vi "Dlg_Settings.vi"(0 "Settings":T1={"Sample Rate (Hz)"=1000.0, "Samples per Channel"=100, "Chassis 1 Channels"="cDAQ1Mod1/ai0:7,cDAQ1Mod2/ai0:7,cDAQ1Mod3/ai0:7,cDAQ1Mod4/ai0:7,cDAQ1Mod5/ai0:7,cDAQ1Mod6/ai0:7,cDAQ1Mod7/ai0:7,cDAQ1Mod8/ai0:7", "Chassis 2 Channels"="cDAQ2Mod1/ai0:7,cDAQ2Mod2/ai0:7,cDAQ2Mod3/ai0:7,cDAQ2Mod4/ai0:7,cDAQ2Mod5/ai0:7,cDAQ2Mod6/ai0:7,cDAQ2Mod7/ai0:7,cDAQ2Mod8/ai0:7", "Save Folder"=path "C:/LV_Test/AI DAQ md test/Data"}, 11 "error in":errorcluster) -> (4 "Settings out":T1={"Sample Rate (Hz)"=1000.0, "Samples per Channel"=100, "Chassis 1 Channels"="cDAQ1Mod1/ai0:7,cDAQ1Mod2/ai0:7,cDAQ1Mod3/ai0:7,cDAQ1Mod4/ai0:7,cDAQ1Mod5/ai0:7,cDAQ1Mod6/ai0:7,cDAQ1Mod7/ai0:7,cDAQ1Mod8/ai0:7", "Chassis 2 Channels"="cDAQ2Mod1/ai0:7,cDAQ2Mod2/ai0:7,cDAQ2Mod3/ai0:7,cDAQ2Mod4/ai0:7,cDAQ2Mod5/ai0:7,cDAQ2Mod6/ai0:7,cDAQ2Mod7/ai0:7,cDAQ2Mod8/ai0:7", "Save Folder"=path "C:/LV_Test/AI DAQ md test/Data"}, 6 "OK?":bool, 15 "error out":errorcluster)   [LabVIEW 2026]
doc: "측정 옵션 팝업: 샘플링 속도, 채널당 샘플 수, 섀시별 물리 채널, 저장 폴더. 확인이면 OK? = True."
panel:
  in  "취소":bool
  in  "확인":bool
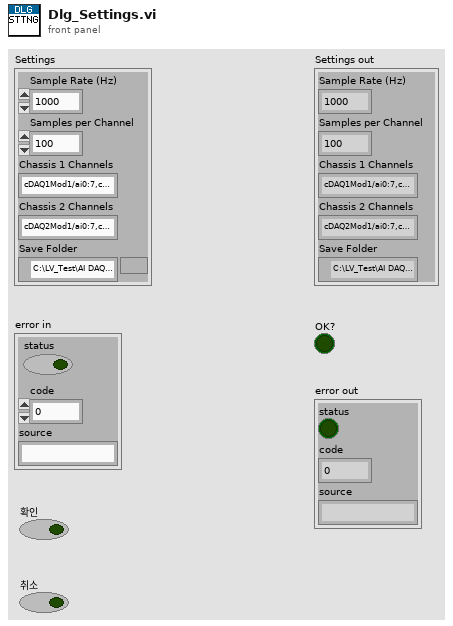
[diagram p1: front panel]
types:
  T1 = cluster{"Sample Rate (Hz)":dbl, "Samples per Channel":i32, "Chassis 1 Channels":string, "Chassis 2 Channels":string, "Save Folder":path}
  T2 = cluster{"Left":i32, "Top":i32, "Right":i32, "Bottom":i32}
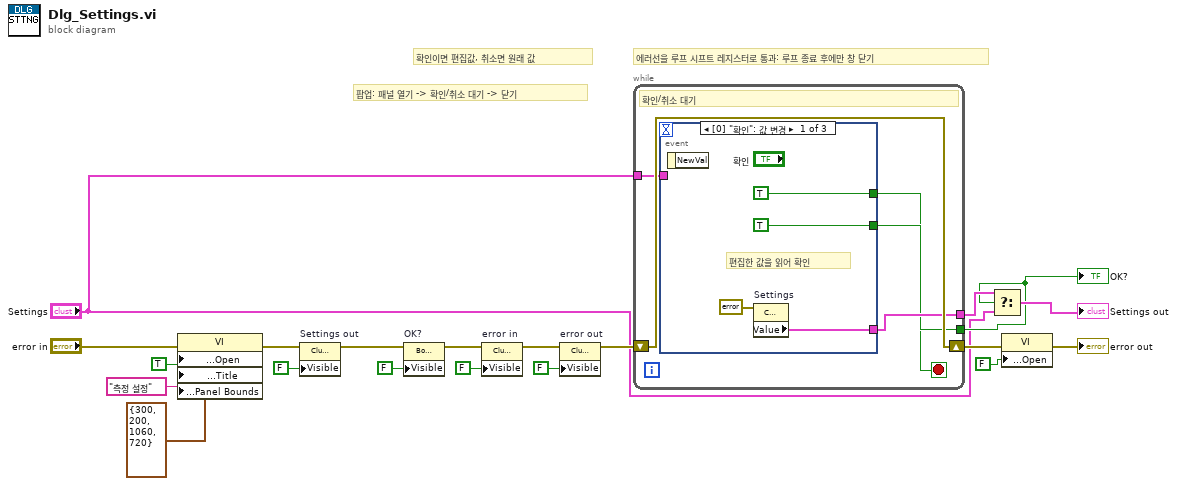
[diagram p0: block diagram]
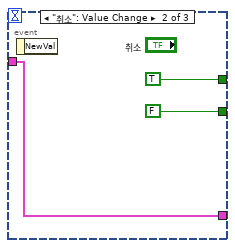
[diagram p2: hidden frame]
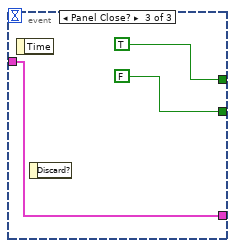
[diagram p3: hidden frame]
diagram:
  # "확인이면 편집값, 취소면 원래 값"
  # "에러선을 루프 시프트 레지스터로 통과: 루프 종료 후에만 창 닫기"
  # "팝업: 패널 열기 -> 확인/취소 대기 -> 닫기"
  n1 = property class="VI"(error in="error in", "Front Panel Window:Open"=TRUE, "Front Panel Window:Title"="측정 설정", "Front Panel Window:Panel Bounds"=T2 {"Left"=300, "Top"=200, "Right"=1060, "Bottom"=720}) -> (error out=w6:errorcluster)  [unwired: 1 in, 1 out]
  n2 = property on="Settings out" class="Clust (엄격한)"(error in=w6, "Visible"=FALSE) -> (error out=w8:errorcluster)  [unwired: 1 in, 1 out]
  n3 = property on="OK?" class="Bool (엄격한)"(error in=w8, "Visible"=FALSE) -> (error out=w10:errorcluster)  [unwired: 1 in, 1 out]
  n4 = property on="error in" class="Clust (엄격한)"(error in=w10, "Visible"=FALSE) -> (error out=w12:errorcluster)  [unwired: 1 in, 1 out]
  n5 = property on="error out" class="Clust (엄격한)"(error in=w12, "Visible"=FALSE) -> (error out=w14:errorcluster)  [unwired: 1 in, 1 out]
  n6 = while {
    tunnel: "Settings" -> [w21]
    tunnel: [w23] -> w15
    tunnel: [w24] -> w16
    shift-right: [w25] -> w17
    shift-left: w14 -> [w25]
    stop <- w22 stop-if-true
    # "확인/취소 대기"
    n7 = event shown="[0] \"확인\": 값 변경" {
      selector: _ -> [_ _ _]
      dyn-events: _ -> [_ _ _]
      timeout: _ -> [_ _ _]
      tunnel: [TRUE TRUE TRUE] -> w22
      tunnel: [TRUE FALSE FALSE] -> w23
      tunnel: w21 -> [_ w30 w33]
      tunnel: [w27 w30 w33] -> w24
      event "확인": Value Change {
        # "편집한 값을 읽어 확인"
        n8 = event-data() -> ()  [unwired: 1 in, 1 out]
        n9 = property on="Settings" class="Clust (엄격한)"(error in=errorcluster {"status"=FALSE, "code"=0, "source"=""}) -> ("Value"=w27:T1)  [unwired: 1 in, 2 out]
      }
      event "취소": Value Change {
        n10 = event-data() -> ()  [unwired: 1 in, 1 out]
      }
      event Panel Close? {
        n11 = event-data() -> ()  [unwired: 1 in, 1 out]
        n12 = event-data() -> ()  [unwired: 2 in, 1 out]
      }
    }
  }
  "OK?" <- w15
  n13 = Select(t=w16, s=w15, f="Settings") -> (s? t:f=→"Settings out":T1)
  n14 = property class="VI"(error in=w17, "Front Panel Window:Open"=FALSE) -> (error out=→"error out":errorcluster)  [unwired: 1 in, 1 out]
